vi "Actor Core.vi"(8 "error in":errorcluster caption="错误输入", 11 "P3AT in":refnum<class "RemoteP3AT.lvclass"> caption="操作者输入") -> (0 "error out":errorcluster caption="错误输出", 3 "Actor out":refnum<class "Actor.lvclass"> caption="操作者输出")   [LabVIEW 2014, in "RemoteP3AT.lvlib" / "RemoteP3AT.lvclass"]
doc: "(<B>文件名</B>：Actor Framework.lvlib:Actor.lvclass:Actor Core.vi)\n\n接收发送至操作者的消息，响应消息并处理可能导致操作者关闭的错误。\n\n子孙类重写该VI，使操作者完成特定的任务。使用调用父方法节点实现重写。"
uses:
  RemoteP3AT.lvclass
  <vilib>/ActorFramework/Actor/Actor.lvclass
  ctl/Point.ctl
  ctl/P3AT_Panel.ctl
  <vilib>/Tufts CEEO ROS for LabVIEW Software/ROS/Code/Console/Servers/ServerSubs/TopicDef.ctl
  <vilib>/Tufts CEEO ROS for LabVIEW Software/ROS/Code/SubVIs/_ROSDirection.ctl
  RemoteP3AT.lvclass/RemoteP3AT.ctl
  <vilib>/ActorFramework/Actor/Actor.lvclass/Actor.ctl
  <vilib>/ActorFramework/Message Enqueuer/Message Enqueuer.lvclass/Message Enqueuer.ctl
  <vilib>/ActorFramework/Message Enqueuer/Enqueue.vi
  Global_var/Global_var.vi
  <vilib>/ActorFramework/Message Priority Queue/Priority Enqueue.vi
  Wrapper_lib/zsActor/ActorWrapper.lvclass
panel:
  out "goal_with_force":T1
  out "vel_set":T2
  out "P3AT_Ini_Pose":T3
  out "P3AT_Panel":T4={"max_vel"=0.49056603773584906, "max_rot"=0.5094339622641509, "Control_Mode"=enum."Joy"} {"max_rot" scale=0.0..1.0; "max_vel" scale=0.0..1.0}
  out "vel_cal":cluster{"rot_z":dbl, "lin_x":dbl}
  out "local_goal":T5
  in  "停止信号":bool
  # "P3AT_Panel 此处不起作用"
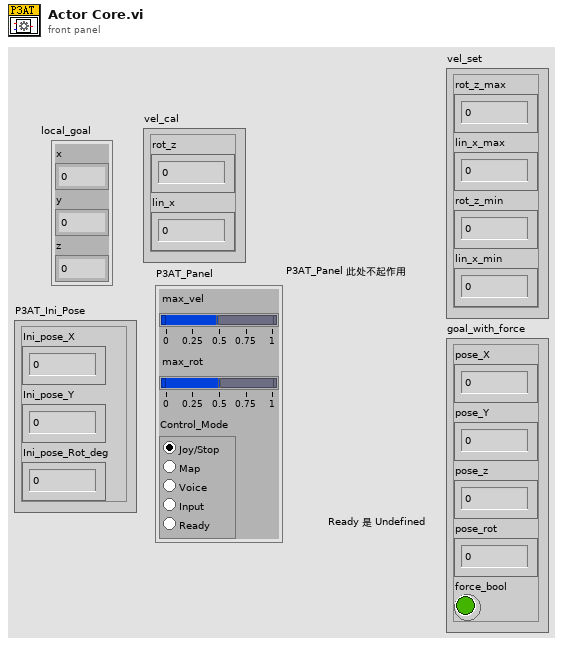
[diagram p1: front panel]
types:
  T1 = cluster{"pose_X":dbl, "pose_Y":dbl, "pose_z":dbl, "pose_rot":dbl, "force_bool":bool}
  T2 = cluster{"rot_z_max":dbl, "lin_x_max":dbl, "rot_z_min":dbl, "lin_x_min":dbl}
  T3 = cluster{"Ini_pose_X":dbl, "Ini_pose_Y":dbl, "Ini_pose_Rot_deg":dbl}
  T4 = typedef "P3AT_Panel.ctl" = cluster{"max_vel":dbl, "max_rot":dbl, "Control_Mode":enum32{"Joy", "Map", "Voice", "Input", "Undefined"}}
  T5 = typedef "Point.ctl" = cluster{"x":dbl, "y":dbl, "z":dbl}
  T6 = typedef "TopicDef.ctl" = cluster{"Topic":string, "Type":string, "Action":T7, "Update (ms)":u16, "queue size":u16}
  T7 = typedef "_ROSDirection.ctl" = enum16{"Node", "Publisher", "Subscriber", "ServiceClient", "ServiceProvider"}
  T8 = typedef "_ROSControl.ctl" = cluster{"topic port":u16, "Node":string, "topic":string, "type":string, "node port":u16, "error ":errorcluster, "Direction":T7, "Update (ms)":u16, "FIFO size":u16}
  T9 = enum32{"Joy", "Map", "Voice", "Input", "Undefined"}
  T10 = typedef "P3AT_Current.ctl" = cluster{"max_vel":dbl, "max_rot":dbl, "now_pose_X":dbl, "now_pose_Y":dbl, "now_pose_Rot_deg":dbl, "Control_Mode":enum32{"Joy", "Map", "Voice", "Input", "Undefined"}}
  T11 = cluster{"now_pose_X":dbl, "now_pose_Y":dbl, "now_pose_Rot_deg":dbl}
  T12 = typedef "Robot_Position.ctl" = cluster{"global x":dbl, "global y":dbl, "global z":dbl, "global_rot":dbl, " floor NO.":dbl}
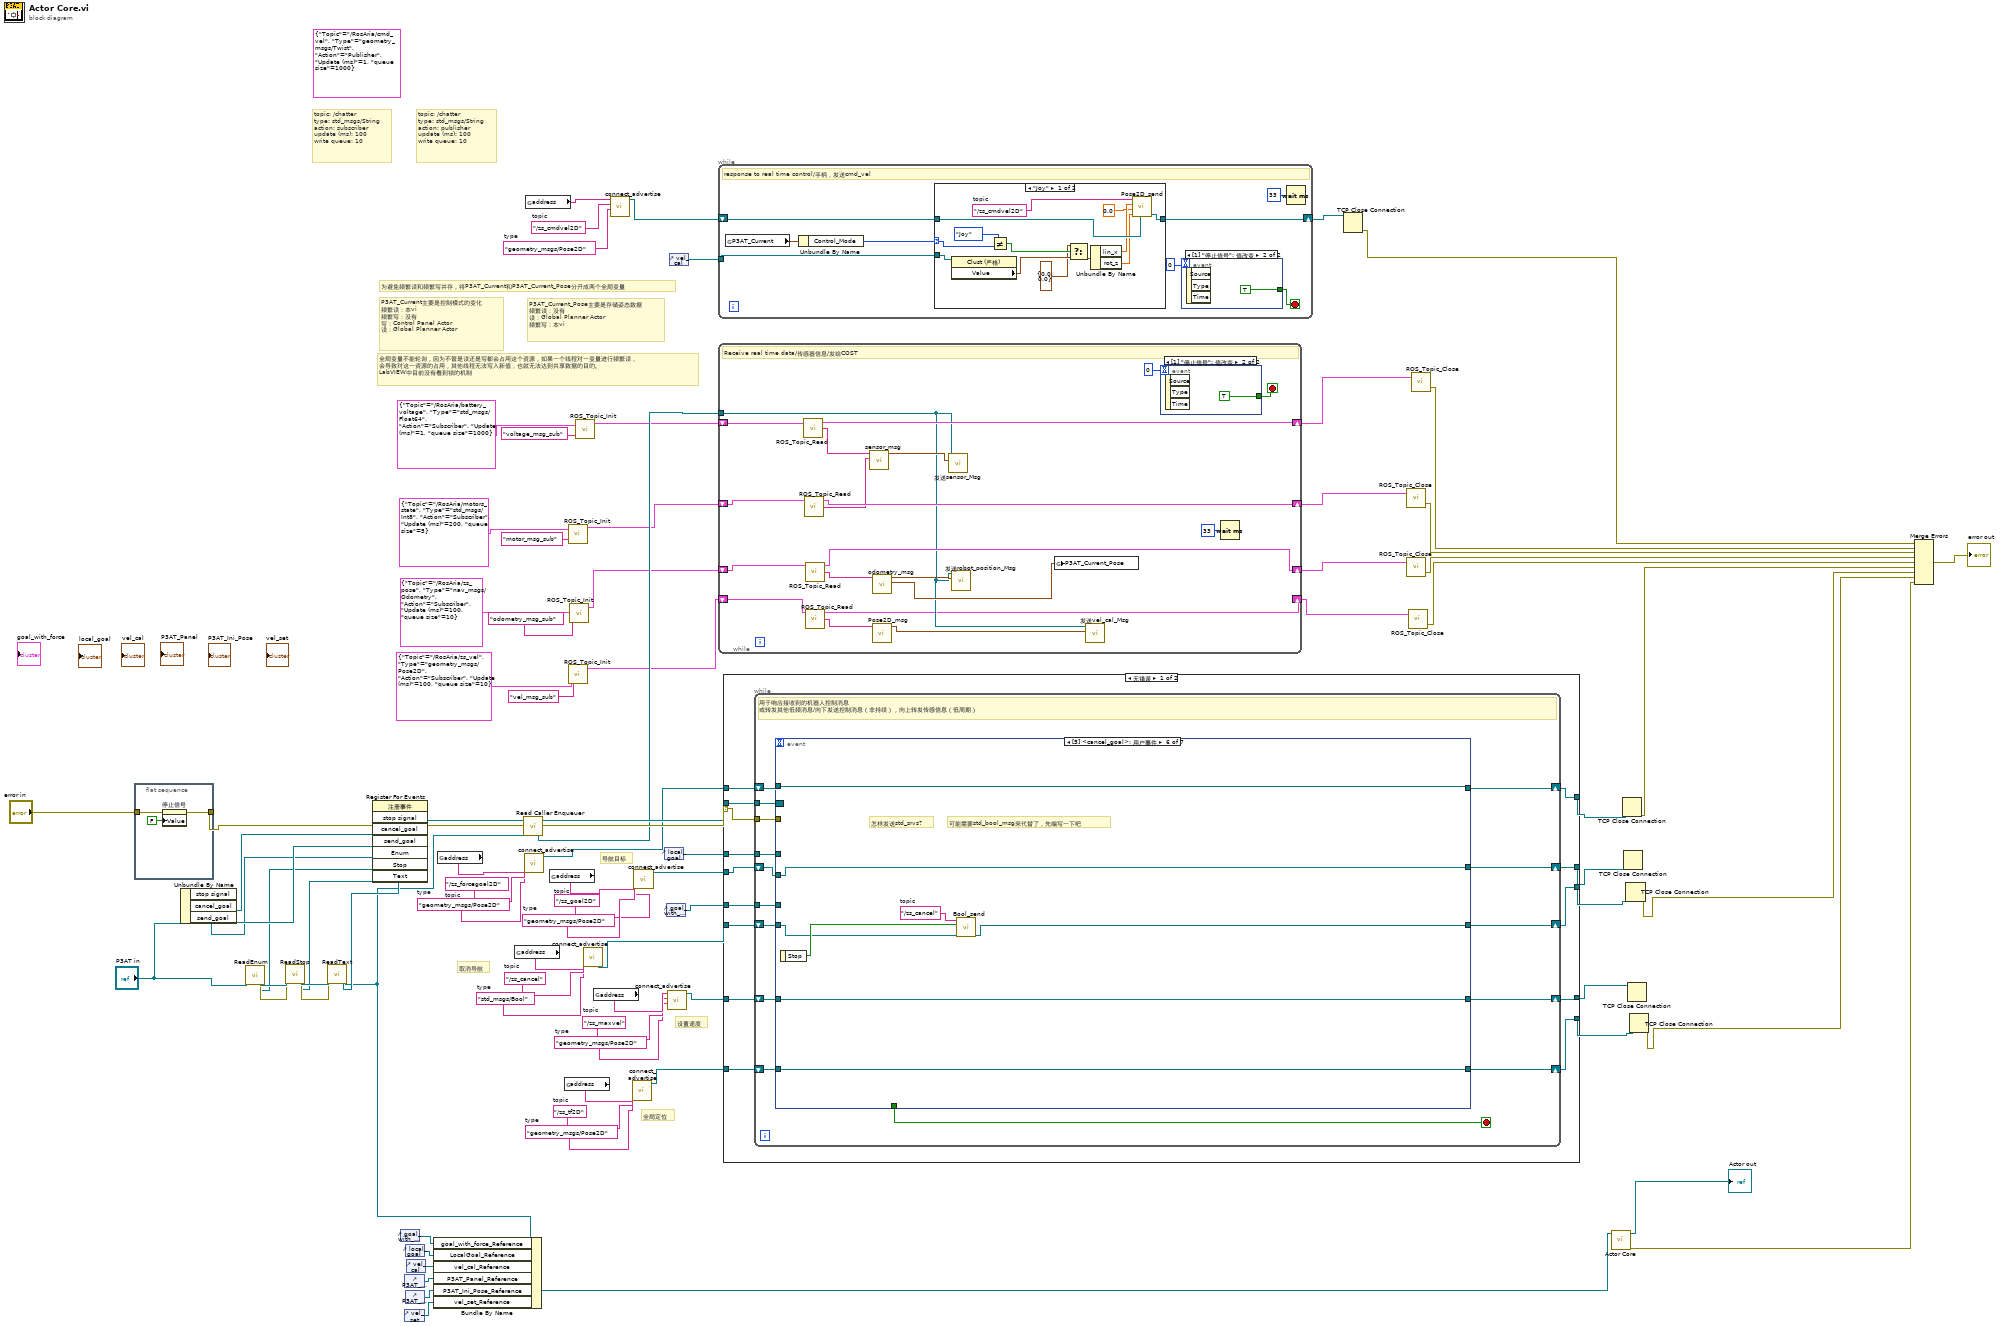
[diagram p0: block diagram]
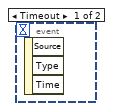
[diagram p3: hidden frame]
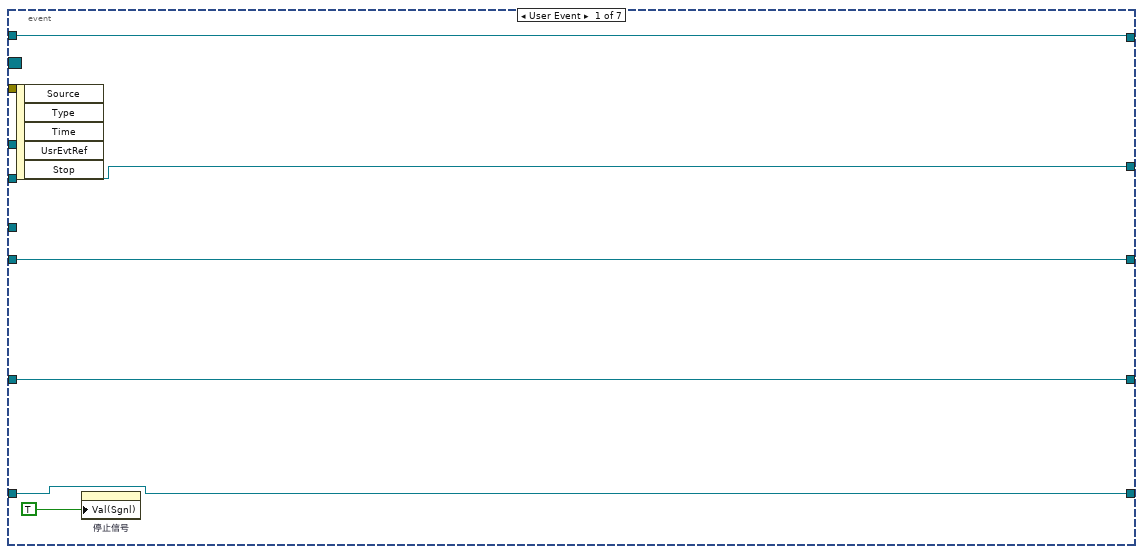
[diagram p4: hidden frame]
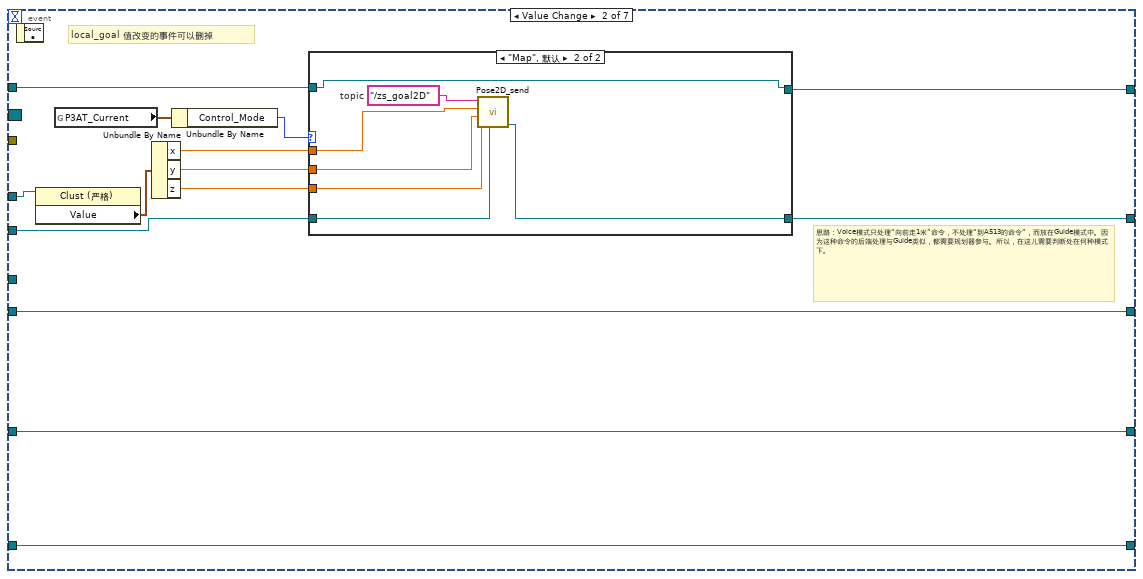
[diagram p5: hidden frame]
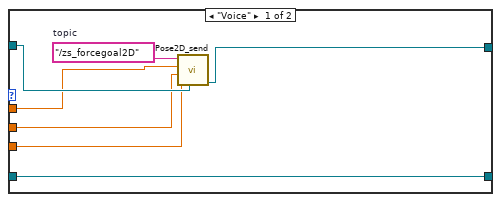
[diagram p6: hidden frame]
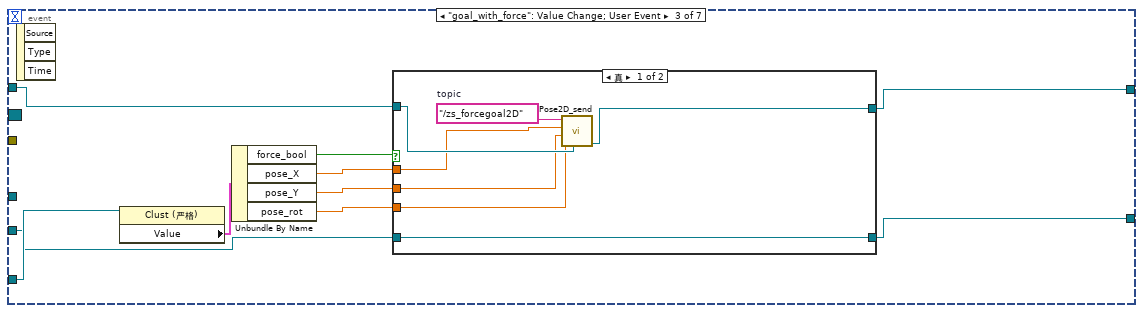
[diagram p7: hidden frame]
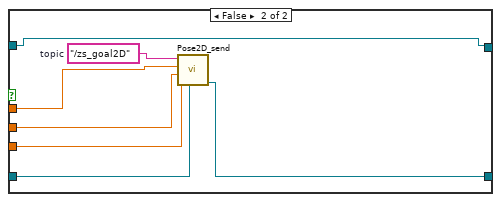
[diagram p8: hidden frame]
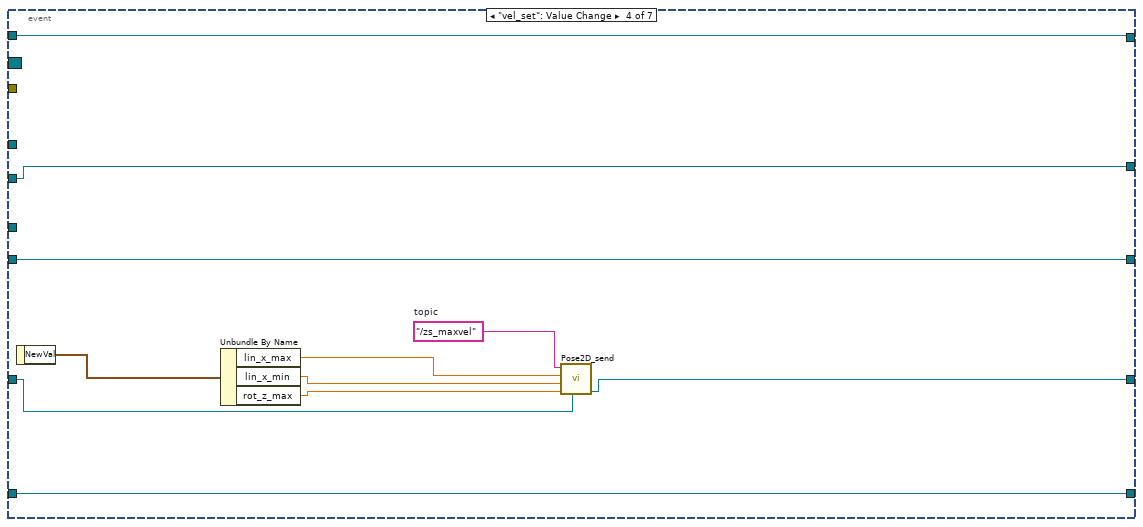
[diagram p9: hidden frame]
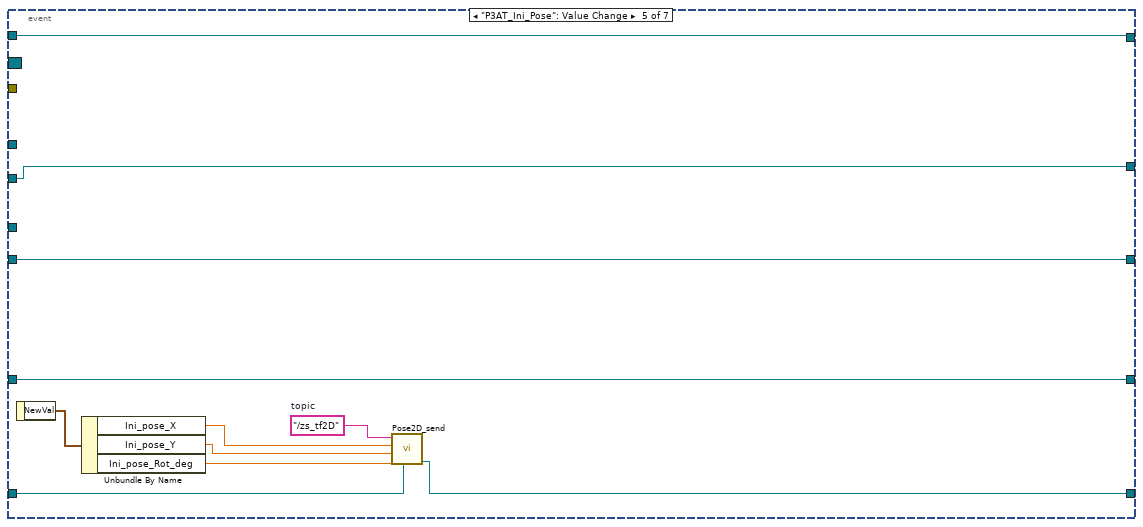
[diagram p10: hidden frame]
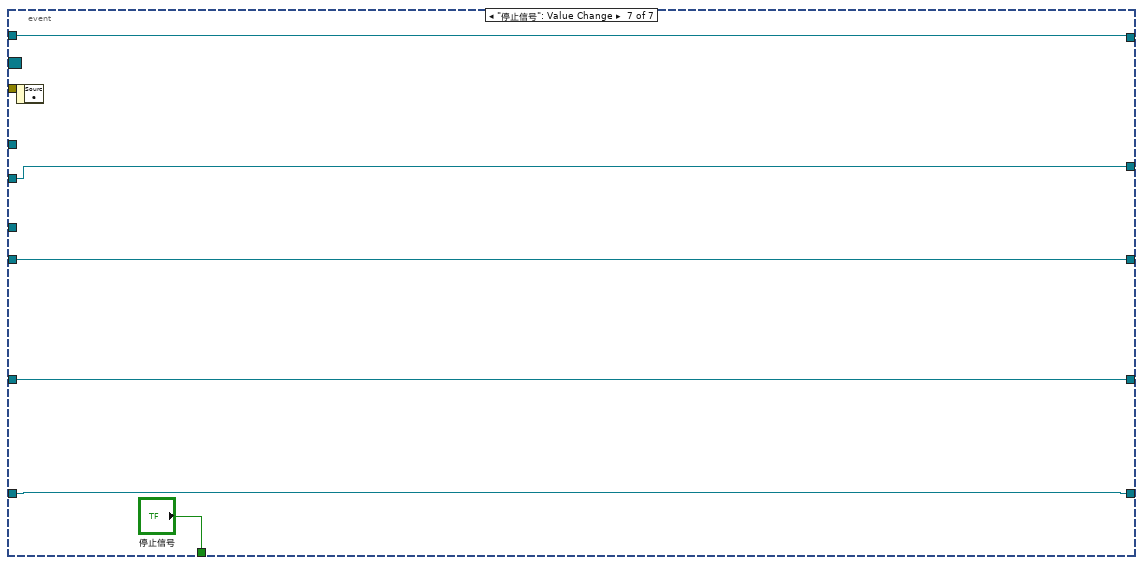
[diagram p11: hidden frame]
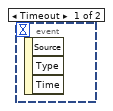
[diagram p13: hidden frame]
diagram:
  w6 = "/zs_maxvel"  # topic
  w5 = "geometry_msgs/Pose2D"  # type
  w19 = "/zs_goal2D"  # topic
  w23 = "geometry_msgs/Pose2D"  # type
  w33 = "/zs_cancel"  # topic
  w32 = "std_msgs/Bool"  # type
  w35 = "/zs_forcegoal2D"  # topic
  w34 = "geometry_msgs/Pose2D"  # type
  w36 = "/zs_tf2D"  # topic
  w37 = "geometry_msgs/Pose2D"  # type
  w41 = "/zs_cmdvel2D"  # topic
  w42 = "geometry_msgs/Pose2D"  # type
  (unwired) T6 {"Topic"="/RosAria/cmd_vel", "Type"="geometry_msgs/Twist", "Action"=enum."Publisher", "Update (ms)"=1, "queue size"=1000} ("Definitions")
  # "设置速度"
  # "全局变量不能轮询，因为不管是读还是写都会占用这个资源，如果一个线程对一变量进行频繁读，\n会导致对这一资源的占用，其他线程无法写入新值，也就无法达到共享数据的目的。\nLabVIEW中目前没有看到锁的机制"
  # "全局定位"
  # "P3AT_Current_Pose主要是存储姿态数据\n频繁读：没有\n读：Global Planner Actor\n频繁写：本vi"
  # "P3AT_Current主要是控制模式的变化\n频繁读：本vi\n频繁写：没有\n写：Control Panel Actor\n读：Global Planner Actor"
  # "为避免频繁读和频繁写并存，将P3AT_Current和P3AT_Current_Pose分开成两个全局变量"
  # "导航目标"
  # "取消导航"
  # "topic: /chatter\ntype: std_msgs/String\naction: subscriber\nupdate (ms): 100\nwrite queue: 10"
  # "topic: /chatter\ntype: std_msgs/String\naction: publisher\nupdate (ms): 100\nwrite queue: 10"
  n1 = flat-sequence {
    tunnel: [w86] -> w80
    tunnel: "error in" -> [w85]
    frame #0 {
      n2 = property on="停止信号" class="Bool (严格)"(error in=w85, "Value"=FALSE ("停止信号")) -> (error out=w86:errorcluster)  [unwired: 1 in, 1 out]
    }
  }
  n3 = Unbundle By Name("P3AT in") -> ("stop signal"=w79:refnum<user-event>, "cancel_goal"=w78:refnum<user-event>, "send_goal"=w43:refnum<user-event>)
  n4 = call-dynamic "ReadEnum.vi"("zsActor输入"="P3AT in") -> ("error out"=w75:errorcluster, "Enum"=w72:refnum<user-event>, "zsActor输出"=w77:refnum<class "RemoteP3AT.lvclass">)  [unwired: 8 in]
  n5 = call-dynamic "ReadStop.vi"("error in (no error)"=w75, "zsActor输入"=w77) -> ("error out"=w74:errorcluster, "Stop"=w71:refnum<user-event>, "zsActor输出"=w76:refnum<class "RemoteP3AT.lvclass">)  [unwired: 7 in]
  n6 = call-dynamic "ReadText.vi"("error in (no error)"=w74, "zsActor输入"=w76) -> ("Text"=w70:refnum<user-event>, "zsActor输出"=w52:refnum<class "RemoteP3AT.lvclass">)  [unwired: 7 in, 1 out]
  n7 = register-events(error in=w80, w79, w78, w43, w72, w71, w70) -> (reference out=w82:refnum<event-registration>, error out=w83:errorcluster)  [unwired: 1 in]
  n8 = control-ref of="goal_with_force"() -> (w2:refnum<vi>)
  n9 = control-ref of="P3AT_Panel"() -> (w47:refnum<vi>)
  n10 = control-ref of="vel_set"() -> (w8:refnum<vi>)
  n11 = control-ref of="local_goal"() -> (w50:refnum<vi>)
  n12 = control-ref of="P3AT_Ini_Pose"() -> (w44:refnum<vi>)
  n13 = control-ref of="vel_cal"() -> (w49:refnum<vi>)
  n14 = Bundle By Name(cluster=w52, "goal_with_force_Reference"=w2, "LocalGoal_Reference"=w50, "vel_cal_Reference"=w49, "P3AT_Panel_Reference"=w47, "P3AT_Ini_Pose_Reference"=w44, "vel_set_Reference"=w8) -> (w51:refnum<class "RemoteP3AT.lvclass">)
  n15 = global read "Global_var.vi" "address"() -> (w20:string)
  n16 = global read "Global_var.vi" "address"() -> (w17:string)
  n17 = call <vilib>:"Read Caller Enqueuer.vi"("Actor"=w52) -> ("Caller Enqueuer"=w69:refnum<class "Message Enqueuer.lvclass">)  [unwired: 10 in]
  n18 = call "connect_advertise.vi"("type"=w34, "topic"=w35, "address"=w20) -> ("连接ID输出"=w31:refnum<k5>)  [unwired: 7 in, 1 out]
  n19 = global read "Global_var.vi" "address"() -> (w15:string)
  n20 = global read "Global_var.vi" "address"() -> (w18:string)
  n21 = global read "Global_var.vi" "address"() -> (w16:string)
  n22 = call <vilib>:"ROS_Topic_Init.vi"("Definitions"=T6 {"Topic"="/RosAria/motors_state", "Type"="std_msgs/Int8", "Action"=enum."Subscriber", "Update (ms)"=200, "queue size"=5}, "node"="motor_msg_sub") -> ("ROS out"=w59:T8)  [unwired: 1 in, 1 out]
  n23 = call <vilib>:"ROS_Topic_Init.vi"("Definitions"=T6 {"Topic"="/RosAria/zs_vel", "Type"="geometry_msgs/Pose2D", "Action"=enum."Subscriber", "Update (ms)"=100, "queue size"=10}, "node"="vel_msg_sub") -> ("ROS out"=w12:T8)  [unwired: 1 in, 1 out]
  n24 = call <vilib>:"ROS_Topic_Init.vi"("Definitions"=T6 {"Topic"="/RosAria/zs_pose", "Type"="nav_msgs/Odometry", "Action"=enum."Subscriber", "Update (ms)"=100, "queue size"=10}, "node"="odometry_msg_sub") -> ("ROS out"=w55:T8)  [unwired: 1 in, 1 out]
  n25 = call <vilib>:"ROS_Topic_Init.vi"("Definitions"=T6 {"Topic"="/RosAria/battery_voltage", "Type"="std_msgs/Float64", "Action"=enum."Subscriber", "Update (ms)"=1, "queue size"=1000}, "node"="voltage_msg_sub") -> ("ROS out"=w61:T8)  [unwired: 1 in, 1 out]
  n26 = call "connect_advertise.vi"("type"=w32, "topic"=w33, "address"=w17) -> ("连接ID输出"=w29:refnum<k5>)  [unwired: 7 in, 1 out]
  n27 = global read "Global_var.vi" "address"() -> (w7:string)
  n28 = call "connect_advertise.vi"("type"=w42, "topic"=w41, "address"=w15) -> ("连接ID输出"=w40:refnum<k5>)  [unwired: 7 in, 1 out]
  n29 = call "connect_advertise.vi"("type"=w37, "topic"=w36, "address"=w16) -> ("连接ID输出"=w25:refnum<k5>)  [unwired: 7 in, 1 out]
  n30 = call "connect_advertise.vi"("type"=w23, "topic"=w19, "address"=w18) -> ("连接ID输出"=w22:refnum<k5>)  [unwired: 7 in, 1 out]
  n31 = control-ref of="local_goal"() -> (w46:refnum<vi>)
  n32 = control-ref of="goal_with_force"() -> (w1:refnum<vi>)
  n33 = call "connect_advertise.vi"("type"=w5, "topic"=w6, "address"=w7) -> ("连接ID输出"=w4:refnum<k5>)  [unwired: 7 in, 1 out]
  n34 = control-ref of="vel_cal"() -> (w48:refnum<vi>)
  n35 = while {
    shift-right: [w91] -> w39
    shift-left: w40 -> [w92]
    tunnel: w48 -> [w90]
    stop <- w94 stop-if-true
    # "response to real time control/手柄，发送cmd_vel"
    n36 = global read "Global_var.vi" "P3AT_Current"() -> (w88:T10)
    n37 = Unbundle By Name(w88) -> ("Control_Mode"=w89:T9)
    n38 = case shown="\"Joy\"" w89 {
      selector: w89 -> [w106 _]
      tunnel: w92 -> [w101 w109]
      tunnel: [w99 w109] -> w91
      tunnel: w90 -> [w108 _]
      frame "Joy" {
        w100 = "/zs_cmdvel2D"  # topic
        n39 = property class="Clust (严格)"(reference=w108) -> ("Value"=w104:cluster{"rot_z":dbl, "lin_x":dbl})  [unwired: 1 in, 2 out]
        n40 = Not Equal?(x=T9."Joy" ("Control_Mode"), y=w106) -> (x != y?=w105:bool)
        n41 = Select(t=cluster{"rot_z":dbl, "lin_x":dbl} {"rot_z"=0.0, "lin_x"=0.0} ("值"), s=w105, f=w104) -> (s? t:f=w102:cluster{"rot_z":dbl, "lin_x":dbl})
        n42 = Unbundle By Name(w102) -> ("lin_x"=w98:dbl, "rot_z"=w96:dbl)
        n43 = call "Pose2D_send.vi"("连接ID"=w101, "msg.theta"=w96, "msg.y"=0.0, "msg.x"=w98, "topic"=w100) -> ("连接ID输出"=w99:refnum<k5>)  [unwired: 6 in]
      }
      frame "Map".."Input", Default {
      }
    }
    n44 = event shown="[1] \"停止信号\": 值改变" {
      selector: _ -> [_ _]
      dyn-events: _ -> [_ _]
      timeout: 0 -> [_ _]
      tunnel: [_ TRUE] -> w94
      event Timeout {
        n45 = event-data() -> ()  [unwired: 1 in, 3 out]
      }
      event "停止信号": Value Change {
        n46 = event-data() -> ()  [unwired: 1 in, 3 out]
      }
    }
    n47 = Wait (ms)(milliseconds to wait=u32 33 ("等待时间（毫秒）")) -> ()  [unwired: 1 out]
  }
  n48 = while {
    tunnel: w69 -> [w115]
    shift-right: [w126] -> w60
    shift-left: w61 -> [w127]
    shift-right: [w124] -> w58
    shift-left: w59 -> [w125]
    shift-right: [w122] -> w54
    shift-left: w55 -> [w123]
    shift-right: [w113] -> w11
    shift-left: w12 -> [w114]
    stop <- w129 stop-if-true
    # "Receive real time data/传感器信息/发给COST"
    n49 = call <vilib>:"ROS_Topic_Read.vi"("ROS in"=w127) -> ("Reply"=w121:string, "ROS out"=w126:T8)  [unwired: 2 in, 1 out]
    n50 = call <vilib>:"ROS_Topic_Read.vi"("ROS in"=w125) -> ("Reply"=w120:string, "ROS out"=w124:T8)  [unwired: 2 in, 1 out]
    n51 = call <vilib>:"ROS_Topic_Read.vi"("ROS in"=w123) -> ("Reply"=w119:string, "ROS out"=w122:T8)  [unwired: 2 in, 1 out]
    n52 = call <vilib>:"ROS_Topic_Read.vi"("ROS in"=w114) -> ("Reply"=w112:string, "ROS out"=w113:T8)  [unwired: 2 in, 1 out]
    n53 = call "sensor_msg.vi"("motor_msg in"=w120, "voltage_msg in"=w121) -> ("sensor_msg_cluster"=w118:cluster{"voltage":dbl, "motor":i8})  [unwired: 9 in]
    n54 = call "Pose2D_msg.vi"("Reply"=w112) -> ("输出簇"=w111:cluster{"rot_z":dbl, "lin_x":dbl})  [unwired: 10 in]
    n55 = call "odometry_msg.vi"("odometry_msg in"=w119) -> ("Current_Pose"=w116:T11, "robot_position_cluster"=w117:T12)  [unwired: 8 in, 1 out]
    n56 = call "发送sensor_Msg.vi"("值(信号)"=w118, "消息待入队列"=w115) -> ()  [unwired: 8 in, 2 out]
    n57 = call "发送robot_position_Msg.vi"("值(信号)"=w117, "消息待入队列"=w115) -> ()  [unwired: 8 in, 2 out]
    n58 = global write "Global_var.vi" "P3AT_Current_Pose"(w116) -> ()
    n59 = call "发送vel_cal_Msg.vi"("值(信号)"=w111, "消息待入队列"=w115) -> ()  [unwired: 8 in, 2 out]
    n60 = event shown="[1] \"停止信号\": 值改变" {
      selector: _ -> [_ _]
      dyn-events: _ -> [_ _]
      timeout: 0 -> [_ _]
      tunnel: [_ TRUE] -> w129
      event Timeout {
        n61 = event-data() -> ()  [unwired: 1 in, 3 out]
      }
      event "停止信号": Value Change {
        n62 = event-data() -> ()  [unwired: 1 in, 3 out]
      }
    }
    n63 = Wait (ms)(milliseconds to wait=u32 33 ("等待时间（毫秒）")) -> ()  [unwired: 1 out]
  }
  n64 = case shown="无错误" w83 {
    selector: w83 -> [w144 _]
    tunnel: w82 -> [w145 _]
    tunnel: [w143 w259] -> w30
    tunnel: [w142 w258] -> w27
    tunnel: w46 -> [w141 _]
    tunnel: [w140 w257] -> w24
    tunnel: w31 -> [w139 w259]
    tunnel: w29 -> [w138 w258]
    tunnel: w25 -> [w137 w257]
    tunnel: w22 -> [w136 w256]
    tunnel: [w135 w256] -> w21
    tunnel: w4 -> [w134 w255]
    tunnel: [w133 w255] -> w3
    tunnel: w1 -> [w132 _]
    frame No Error {
      n65 = while {
        tunnel: w145 -> [w160]
        tunnel: w144 -> [w158]
        shift-right: [w157] -> w143
        shift-left: w139 -> [w156]
        shift-right: [w154] -> w142
        shift-left: w138 -> [w155]
        tunnel: w141 -> [w153]
        shift-right: [w151] -> w140
        shift-left: w137 -> [w152]
        shift-right: [w149] -> w135
        shift-left: w136 -> [w150]
        shift-right: [w147] -> w133
        shift-left: w134 -> [w148]
        tunnel: w132 -> [w146]
        stop <- w159 stop-if-true
        # "用于响应接收到的机器人控制消息\n或转发其他低频消息/向下发送控制消息（非持续），向上转发传感信息（低周期）"
        n66 = event shown="[5] <cancel_goal>: 用户事件" {
          selector: w160 -> [_ _ _ _ _ _ _]
          dyn-events: _ -> [_ _ _ _ _ _ _]
          timeout: _ -> [_ _ _ _ _ _ _]
          tunnel: [_ _ _ _ _ _ "停止信号"] -> w159
          tunnel: w158 -> [_ _ _ _ _ _ _]
          tunnel: w156 -> [w165 w174 w198 w222 w238 w248 w253]
          tunnel: [w165 w170 w196 w222 w238 w248 w253] -> w157
          tunnel: w155 -> [w164 w180 _ w220 w239 w244 w252]
          tunnel: [w164 w180 _ w220 w239 w243 w252] -> w154
          tunnel: w153 -> [_ w179 _ _ _ _ _]
          tunnel: w152 -> [w163 w177 _ w219 w237 w247 w251]
          tunnel: [w163 w177 _ w219 w236 w247 w251] -> w151
          tunnel: w150 -> [w162 w169 w197 w221 w231 w242 w250]
          tunnel: [w162 w168 w195 w221 w231 w242 w250] -> w149
          tunnel: w148 -> [w161 w167 _ w224 w230 w241 w249]
          tunnel: [w161 w167 _ w223 w230 w241 w249] -> w147
          tunnel: w146 -> [_ _ w200 _ _ _ _]
          event User Event {
            n67 = event-data() -> ()  [unwired: 1 in, 5 out]
            n68 = property on="停止信号" class="Bool (严格)"("Val(Sgnl)"=TRUE ("值(信号)")) -> ()  [unwired: 2 in, 2 out]
          }
          event Value Change {
            # "思路：Voice模式只处理“向前走1米”命令，不处理“到A513的命令”，而放在Guide模式中。因为这种命令的后端处理与Guide类似，都需要规划器参与。所以，在这儿需要判断处在何种模式下。"
            # "local_goal 值改变的事件可以删掉"
            n69 = event-data() -> ()  [unwired: 1 in, 1 out]
            n70 = property class="Clust (严格)"(reference=w179) -> ("Value"=w178:T5)  [unwired: 1 in, 2 out]
            n71 = global read "Global_var.vi" "P3AT_Current"() -> (w176:T10)
            n72 = Unbundle By Name(w178) -> ("x"=w173:dbl, "y"=w172:dbl, "z"=w171:dbl)
            n73 = Unbundle By Name(w176) -> ("Control_Mode"=w175:T9)
            n74 = case shown="\"Map\", 默认" w175 {
              tunnel: w174 -> [w187 w188]
              tunnel: w173 -> [w185 w193]
              tunnel: w172 -> [w184 w192]
              tunnel: w171 -> [w183 w191]
              tunnel: [w182 w188] -> w170
              tunnel: w169 -> [w181 w190]
              tunnel: [w181 w189] -> w168
              frame "Voice" {
                w186 = "/zs_forcegoal2D"  # topic
                n75 = call "Pose2D_send.vi"("连接ID"=w187, "msg.theta"=w183, "msg.y"=w184, "msg.x"=w185, "topic"=w186) -> ("连接ID输出"=w182:refnum<k5>)  [unwired: 6 in]
              }
              frame "Map", Default {
                w194 = "/zs_goal2D"  # topic
                n76 = call "Pose2D_send.vi"("连接ID"=w190, "msg.theta"=w191, "msg.y"=w192, "msg.x"=w193, "topic"=w194) -> ("连接ID输出"=w189:refnum<k5>)  [unwired: 6 in]
              }
            }
          }
          event "goal_with_force": Value Change; User Event {
            n77 = event-data() -> ()  [unwired: 1 in, 3 out]
            n78 = property class="Clust (严格)"(reference=w200) -> ("Value"=w201:T1)  [unwired: 1 in, 2 out]
            n79 = Unbundle By Name(w201) -> ("force_bool"=w199:bool, "pose_X"=w202:dbl, "pose_Y"=w203:dbl, "pose_rot"=w204:dbl)
            n80 = case shown="真" w199 {
              tunnel: w198 -> [w211 w212]
              tunnel: w202 -> [w209 w217]
              tunnel: w203 -> [w208 w216]
              tunnel: w204 -> [w207 w215]
              tunnel: [w206 w212] -> w196
              tunnel: w197 -> [w205 w214]
              tunnel: [w205 w213] -> w195
              frame True {
                w210 = "/zs_forcegoal2D"  # topic
                n81 = call "Pose2D_send.vi"("连接ID"=w211, "msg.theta"=w207, "msg.y"=w208, "msg.x"=w209, "topic"=w210) -> ("连接ID输出"=w206:refnum<k5>)  [unwired: 6 in]
              }
              frame False {
                w218 = "/zs_goal2D"  # topic
                n82 = call "Pose2D_send.vi"("连接ID"=w214, "msg.theta"=w215, "msg.y"=w216, "msg.x"=w217, "topic"=w218) -> ("连接ID输出"=w213:refnum<k5>)  [unwired: 6 in]
              }
            }
          }
          event "vel_set": Value Change {
            w228 = "/zs_maxvel"  # topic
            n83 = event-data() -> ("NewVal"=w229:T2)  [unwired: 1 in]
            n84 = Unbundle By Name(w229) -> ("lin_x_max"=w227:dbl, "lin_x_min"=w226:dbl, "rot_z_max"=w225:dbl)
            n85 = call "Pose2D_send.vi"("连接ID"=w224, "msg.theta"=w225, "msg.y"=w226, "msg.x"=w227, "topic"=w228) -> ("连接ID输出"=w223:refnum<k5>)  [unwired: 6 in]
          }
          event "P3AT_Ini_Pose": Value Change {
            w235 = "/zs_tf2D"  # topic
            n86 = event-data() -> ("NewVal"=w240:T3)  [unwired: 1 in]
            n87 = Unbundle By Name(w240) -> ("Ini_pose_X"=w234:dbl, "Ini_pose_Y"=w233:dbl, "Ini_pose_Rot_deg"=w232:dbl)
            n88 = call "Pose2D_send.vi"("连接ID"=w237, "msg.theta"=w232, "msg.y"=w233, "msg.x"=w234, "topic"=w235) -> ("连接ID输出"=w236:refnum<k5>)  [unwired: 6 in]
          }
          event User Event {
            w245 = "/zs_cancel"  # topic
            # "可能需要std_bool_msg来代替了，先编写一下吧"
            # "怎样发送std_srvs?"
            n89 = event-data() -> ("Stop"=w246:bool)  [unwired: 1 in]
            n90 = call "Bool_send.vi"("连接ID"=w244, "msg.data"=w246, "topic"=w245) -> ("连接ID输出"=w243:refnum<k5>)  [unwired: 8 in]
          }
          event "停止信号": Value Change {
            n91 = event-data() -> ()  [unwired: 1 in, 1 out]
          }
        }
      }
    }
    frame Error {
    }
  }
  n92 = TCP Close Connection(connection ID=w39) -> (error out=w38:errorcluster)  [unwired: 2 in, 1 out]
  n93 = call <vilib>:"ROS_Topic_Close.vi"("ROS in"=w58) -> ("error out"=w63:errorcluster)  [unwired: 3 in]
  n94 = call <vilib>:"ROS_Topic_Close.vi"("ROS in"=w54) -> ("error out"=w53:errorcluster)  [unwired: 3 in]
  n95 = call <vilib>:"ROS_Topic_Close.vi"("ROS in"=w11) -> ("error out"=w9:errorcluster)  [unwired: 3 in]
  n96 = call <vilib>:"ROS_Topic_Close.vi"("ROS in"=w60) -> ("error out"=w62:errorcluster)  [unwired: 3 in]
  n97 = call-parent "Actor Core.vi"("Actor in"=w51) -> ("error out"=w45:errorcluster, "Actor out"=→"Actor out":refnum<class "Actor.lvclass">)  [unwired: 9 in]
  n98 = TCP Close Connection(connection ID=w30) -> (error out=w10:errorcluster)  [unwired: 2 in, 1 out]
  n99 = TCP Close Connection(connection ID=w21) -> ()  [unwired: 2 in, 2 out]
  n100 = TCP Close Connection(connection ID=w27) -> (error out=w28:errorcluster)  [unwired: 2 in, 1 out]
  n101 = TCP Close Connection(connection ID=w3) -> ()  [unwired: 2 in, 2 out]
  n102 = TCP Close Connection(connection ID=w24) -> (error out=w26:errorcluster)  [unwired: 2 in, 1 out]
  n103 = Merge Errors(w38, w62, w63, w53, w9, w10, w28, w26, w45) -> (→"error out":errorcluster)
